vi "init.vi"(8 "error in":errorcluster, 10 "TBM module configuration in":refnum<class "TBM module configuration.lvclass">, 11 "TEC runtime in":refnum<class "TEC runtime.lvclass">) -> (0 "error out":errorcluster, 1 "data allocations":T1, 2 "execution settings":T4, 3 "TEC runtime out":refnum<class "TEC runtime.lvclass">)   [LabVIEW 2013, in "TEC runtime.lvclass"]
doc: "Provides an interface for initializing a module at runtime. While this interface performs no operations, a child should provide an override which may open any necessary references or sessions, allocate necessary memory, and perform any final configuration validataion before providing the full configuration <b>execution data</b> to the calling process."
uses:
  TEC runtime.lvclass
  <vilib>/NI/Tag Bus Module Framework/module configuration/TBM module configuration.lvclass
  <vilib>/NI/Tag Bus Module Framework/runtime/execution settings.ctl
  <vilib>/NI/Tag Bus Module Framework/channel/data tables.ctl
  <vilib>/NI/Tag Bus/dictionary/data dictionary.lvclass
  <vilib>/NI/Tag Bus/dictionary table pair.ctl
  <vilib>/NI/Tag Bus/table/data table.ctl
  configuration/TEC configuration.lvclass
  configuration/TEC configuration.lvclass/TEC configuration.ctl
  TEC runtime.lvclass/TEC runtime.ctl
  configuration/Read send to address.vi
  configuration/Read send to port.vi
  configuration/Read receive on port.vi
  configuration/Read send from port.vi
  configuration/Read estimated array size.vi
  <vilib>/NI/Tag Bus Module Framework/channel/TBM channel.lvclass
  <vilib>/NI/Tag Bus Module Framework/runtime/TBM module execution interface.lvclass
  <vilib>/NI/Tag Bus/tag bus.lvlib
  <vilib>/NI/Tag Bus/table/data table.lvlib
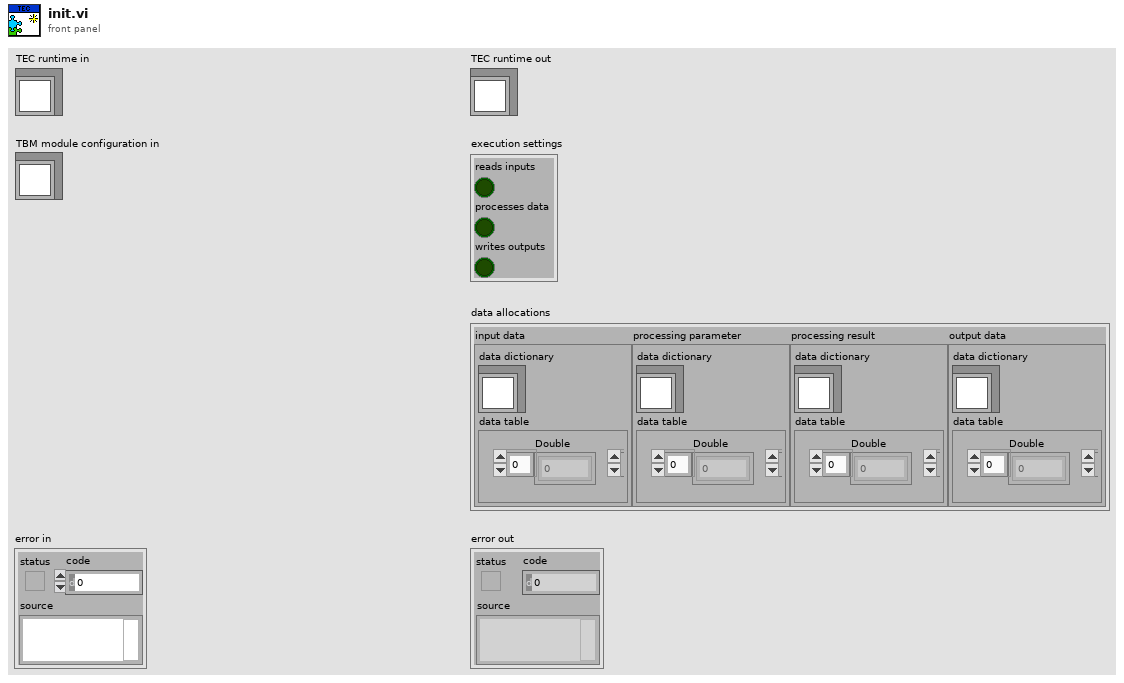
[diagram p1: front panel]
types:
  T1 = typedef "TBM channel.lvclass/data tables.ctl" = cluster{"input data":T2, "processing parameter":T2, "processing result":T2, "output data":T2}
  T2 = typedef "tag bus.lvlib/dictionary table pair.ctl" = cluster{"data dictionary":refnum<class "data dictionary.lvclass">, "data table":T3}
  T3 = typedef "tag bus.lvlib/data table.lvlib/data table.ctl" = cluster{"Double":dbl[], "Single":sgl[], "I64":i64[], "I32":i32[], "I16":i16[], "I8":i8[], "U64":u64[], "U32":u32[], "U16":u16[], "U8":u8[], "Boolean":bool[], "String":string[], "Array of Double":cluster{"DBL Array":dbl[]}[], "Array of Single":cluster{"SGL Array":sgl[]}[], "Array of I64":cluster{"I64 Array":i64[]}[], "Array of I32":cluster{"I32 Array":i32[]}[], "Array of I16":cluster{"I16 Array":i16[]}[], "Array of I8":cluster{"I8 Array":i8[]}[], "Array of U64":cluster{"U64 Array":u64[]}[], "Array of U32":cluster{"U32 Array":u32[]}[], "Array of U16":cluster{"U16 Array":u16[]}[], "Array of U8":cluster{"U8 Array":u8[]}[], "Array of Boolean":cluster{"Boolean Array":bool[]}[], "Array of String":cluster{"String Array":string[]}[]}
  T4 = typedef "TBM module execution interface.lvclass/execution settings.ctl" = cluster{"reads inputs":bool, "processes data":bool, "writes outputs":bool}
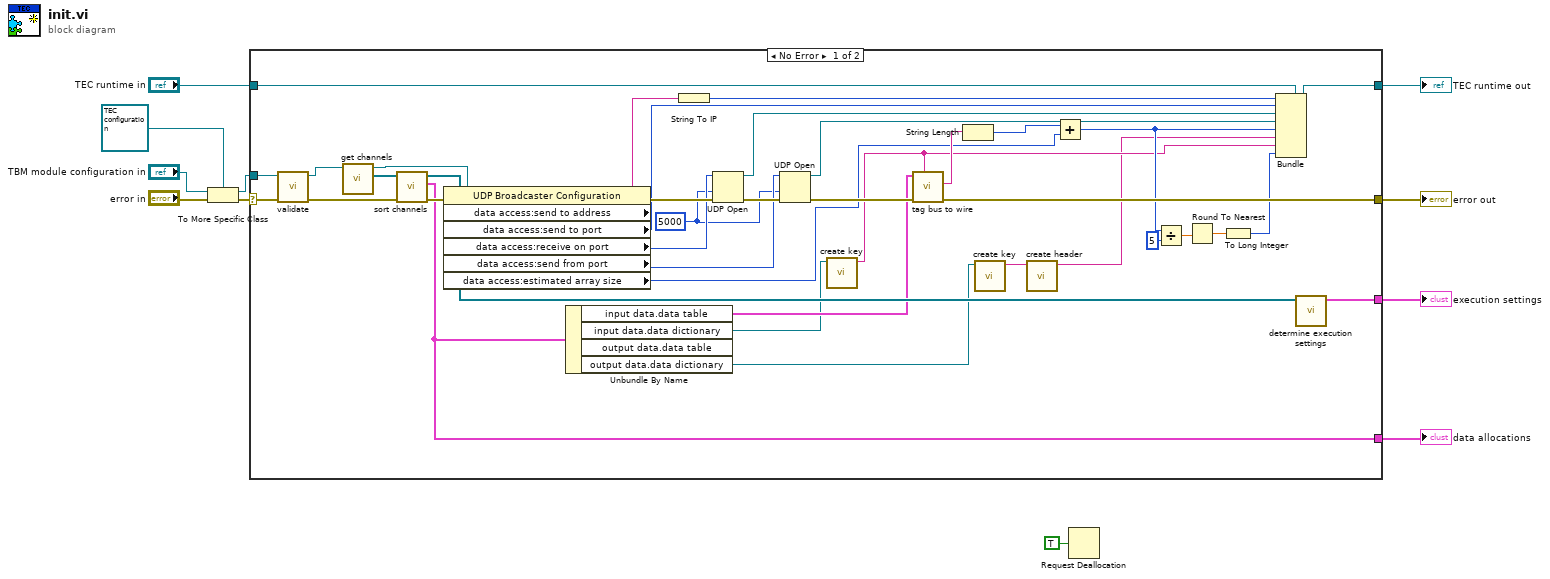
[diagram p0: block diagram]
diagram:
  n1 = To More Specific Class(target class=refnum<class "TEC configuration.lvclass"> refnum ("TEC configuration"), reference="TBM module configuration in", error in="error in") -> (specific class reference=w10:refnum<class "TEC configuration.lvclass">, error out=w11:errorcluster)
  n2 = case shown="No Error" w11 {
    selector: w11 -> [w45 w50]
    tunnel: w10 -> [w41 _]
    tunnel: "TEC runtime in" -> [w49 w51]
    tunnel: [w42 w51] -> w2
    tunnel: [w25 w50] -> w6
    tunnel: [w26 _] -> w4
    tunnel: [w48 _] -> w5
    frame No Error {
      w29 = 5000 ("timeout ms (25000)")
      n3 = call-dynamic "validate.vi"("error in"=w45, "TEC configuration in"=w41) -> ("error out"=w46:errorcluster, "TEC configuration out"=w44:refnum<class "TEC configuration.lvclass">)  [unwired: 8 in]
      n4 = call-dynamic "get channels.vi"("TEC configuration in"=w44) -> ("channels"=w43:refnum<class "TBM channel.lvclass">[], "TEC configuration out"=w38:refnum<class "TEC configuration.lvclass">)  [unwired: 9 in]
      n5 = call <vilib>:"sort channels.vi"("error in"=w46, "channels in"=w43) -> ("error out"=w40:errorcluster, "data allocations"=w26:T1, "channels out"=w47:refnum<class "TBM channel.lvclass">[])  [unwired: 7 in]
      n6 = property class="UDP Broadcaster Configuration"(reference=w38, error in=w40) -> (error out=w39:errorcluster, "data access:send to address"=w35:string, "data access:send to port"=w37:u16, "data access:receive on port"=w30:u16, "data access:send from port"=w31:u16, "data access:estimated array size"=w16:u16)  [unwired: 1 out]
      n7 = Unbundle By Name(w26) -> ("input data.data table"=w24:T3, "input data.data dictionary"=w22:refnum<class "data dictionary.lvclass">, "output data.data dictionary"=w23:refnum<class "data dictionary.lvclass">)  [unwired: 1 out]
      n8 = String To IP(1:w35) -> (0:w36:u32)
      n9 = UDP Open(8:w39, 9:w29, 11:w30) -> (port=w32:refnum<k16>, 0:w34:errorcluster)  [unwired: 2 in, 1 out]
      n10 = UDP Open(8:w34, 9:w29, 11:w31) -> (port=w33:refnum<k16>, 0:w27:errorcluster)  [unwired: 2 in, 1 out]
      n11 = call "create key.vi"("data dictionary in"=w22) -> ("key"=w14:string)  [unwired: 10 in]
      n12 = call "tag bus to wire.vi"("unique key"=w14, "error in"=w27, "data table in"=w24) -> ("error out"=w25:errorcluster, "wire data"=w28:string)  [unwired: 5 in, 2 out]
      n13 = String Length(string=w28) -> (length=w21:i32)
      n14 = call "create key.vi"("data dictionary in"=w23) -> ("key"=w13:string)  [unwired: 10 in]
      n15 = call "create header.vi"("unique key"=w13) -> ("wire data"=w12:string)  [unwired: 10 in]
      n16 = Add(x=w21, y=w16) -> (x+y=w17:i32)
      n17 = Divide(x=w17, y=5) -> (x/y=w19:dbl)
      n18 = Round To Nearest(number=w19) -> (nearest integer value=w18:dbl)
      n19 = To Long Integer(number=w18) -> (32bit integer=w15:i32)
      n20 = Bundle(cluster=w49, w36, w37, w32, w33, w17, w12, w14, w15) -> (w42:refnum<class "TEC runtime.lvclass">)
      n21 = call <vilib>:"determine execution settings.vi"("channels"=w47) -> ("execution settings"=w48:T4)  [unwired: 10 in]
    }
    frame Error {
    }
  }
  "error out" <- w6
  "TEC runtime out" <- w2
  "execution settings" <- w5
  "data allocations" <- w4
  n22 = Request Deallocation(TRUE ("flag")) -> ()
